vi "Write Setting.vi"(8 "error in (no error)":errorcluster, 10 "Setting":T1={"Local Database"="JungDB", "Connect OPC Trial"=0, "Timeout Connect OPC"=0.0, "AbstractUUT Path"="C:\\Working copy\\TS Manager\\Plugin\\Tests\\Submodule EOL\\TS Execution Interface\\OPC UA\\Abstract.lvclass", "PreUUT Path"="C:\\Working copy\\TS Manager\\Plugin\\Tests\\Submodule EOL\\TS Execution Interface\\PreUUT\\PreUUT.lvclass", "Test Path"="C:\\Working copy\\TS Manager\\Plugin\\Tests\\Submodule EOL\\TS Execution Interface\\TestExec\\TestExec.lvclass", "PostUUT Path"="C:\\Working copy\\TS Manager\\Plugin\\Tests\\Submodule EOL\\TS Execution Interface\\PostUUT\\PostUUT.lvclass"} {"Timeout Connect OPC" format="%#_f"}, 11 "Submodule EOL configuration":refnum<class "Submodule EOL configuration.lvclass">) -> (0 "error out":errorcluster, 3 "Submodule EOL configuration out":refnum<class "Submodule EOL configuration.lvclass">)   [LabVIEW 2025, in "Submodule EOL.lvlib" / "Submodule EOL configuration.lvclass"]
uses:
  Submodule EOL configuration.lvclass
  Setting.ctl
  Submodule EOL configuration.lvclass/Submodule EOL configuration.ctl
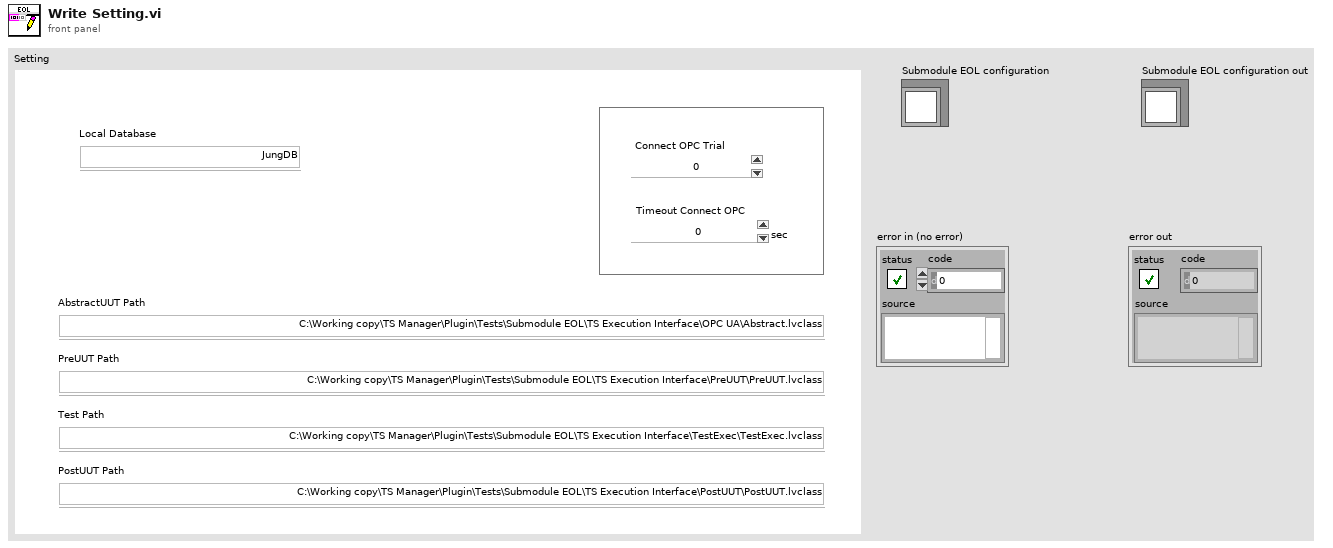
[diagram p1: front panel]
types:
  T1 = typedef "Submodule EOL.lvlib/Submodule EOL configuration.lvclass/Setting.ctl" = cluster{"Local Database":string, "Connect OPC Trial":u32, "Timeout Connect OPC":dbl, "AbstractUUT Path":string, "PreUUT Path":string, "Test Path":string, "PostUUT Path":string}
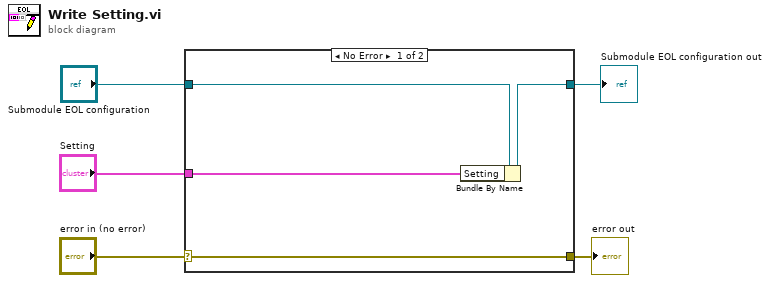
[diagram p0: block diagram]
diagram:
  n1 = case shown="No Error" "error in (no error)" {
    selector: "error in (no error)" -> [w9 w10]
    tunnel: [w9 w10] -> w4
    tunnel: [w7 w11] -> w1
    tunnel: "Submodule EOL configuration" -> [w8 w11]
    tunnel: "Setting" -> [w6 _]
    frame No Error {
      n2 = Bundle By Name(cluster=w8, "Setting"=w6) -> (w7:refnum<class "Submodule EOL configuration.lvclass">)
    }
    frame Error {
    }
  }
  "error out" <- w4
  "Submodule EOL configuration out" <- w1
